vi "detect modules.vi"() -> (0 "error out":errorcluster, 1 "device models":string[](array[string]), 2 "passed?":bool)   [LabVIEW 2014, in "tests.lvlib"]
uses:
  tests.lvlib
  classes/Device/FG action.ctl
  classes/SysCfg Device/SysCfg Device.lvclass
  classes/Controller/Controller.lvclass
  classes/Chassis/Chassis.lvclass
  classes/Device/Device.lvclass
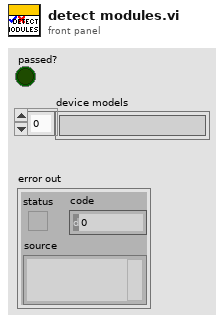
[diagram p1: front panel]
types:
  T1 = typedef "SMI.lvlib/Device.lvclass/FG action.ctl" = enum16{"get", "set"}
  T2 = typedef "SMI.lvlib/Device.lvclass/login credentials.ctl" = cluster{"device class":string, "hostname":string, "IP address":string, "username":string, "password":string}
  T3 = typedef "SMI.lvlib/Chassis.lvclass/chassis and module information.ctl" = cluster{"chassis":T4, "modules":T5[]}
  T4 = typedef "SMI.lvlib/Chassis.lvclass/chassis information.ctl" = cluster{"resource name":string, "vendor name":string, "product name":string, "product ID":u16, "serial number":string, "number of slots":i32, "device class":string}
  T5 = typedef "SMI.lvlib/Module.lvclass/module information.ctl" = cluster{"vendor name":string, "product name":string, "product ID":u16, "serial number":string}
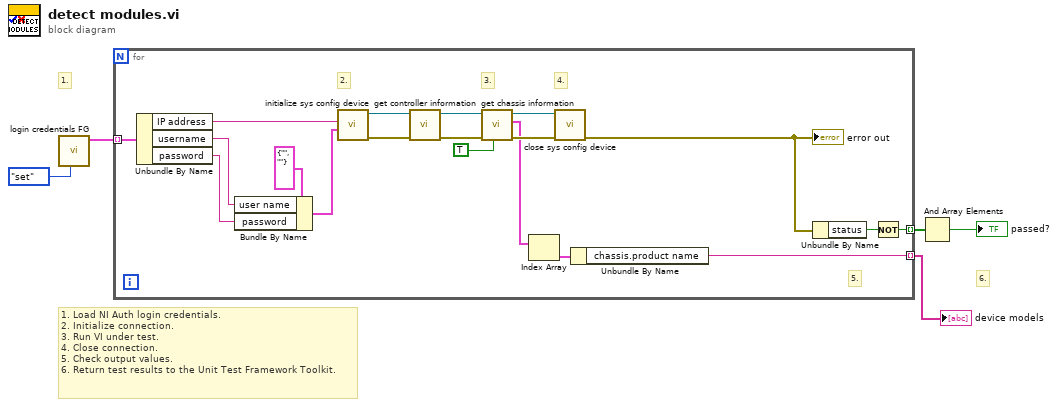
[diagram p0: block diagram]
diagram:
  # "1."
  # "6."
  # "1. Load NI Auth login credentials.\n2. Initialize connection.\n3. Run VI under test.\n4. Close connection.\n5. Check output values.\n6. Return test results to the Unit Test Framework Toolkit."
  n1 = call "login credentials FG.vi"("FG action"=FG_action."set") -> ("login credentials"=w3:T2[])  [unwired: 9 in, 1 out]
  n2 = for {
    tunnel: [w22] -> w4 mode=indexing
    tunnel: w3 -> [w13] mode=indexing
    tunnel: [w6] -> w2 mode=indexing
    # "4."
    # "2."
    # "3."
    # "5."
    n3 = Unbundle By Name(w13) -> ("IP address"=w12:string, "username"=w10:string, "password"=w11:string)
    n4 = Bundle By Name(cluster=cluster{"user name":string, "password":string} {"user name"="", "password"=""} ("login"), "user name"=w10, "password"=w11) -> (w14:cluster{"user name":string, "password":string})
    n5 = call "initialize sys config device.vi"("login"=w14, "IP address (localhost)"=w12) -> ("error out"=w24:errorcluster, "controller out"=w23:refnum<class "Controller.lvclass">)  [unwired: 8 in]
    n6 = call "get controller information.vi"("error in"=w24, "controller in"=w23) -> ("error out"=w21:errorcluster, "controller out"=w19:refnum<class "Controller.lvclass">)  [unwired: 7 in, 1 out]
    n7 = call "get chassis information.vi"("detect modules (T)"=TRUE, "error in"=w21, "controller in"=w19) -> ("error out"=w20:errorcluster, "local chassis"=w8:T3[], "controller out"=w18:refnum<class "Controller.lvclass">)  [unwired: 5 in, 1 out]
    n8 = Index Array(array=w8) -> (element=w7:T3)  [unwired: 1 in]
    n9 = call "close sys config device.vi"("error in"=w20, "controller in"=w18) -> ("error out"=w9:errorcluster)  [unwired: 8 in, 1 out]
    "error out" <- w9
    n10 = Unbundle By Name(w7) -> ("chassis.product name"=w6:string)
    n11 = Unbundle By Name(w9) -> ("status"=w17:bool)
    n12 = Not(x=w17) -> (.not. x?=w22:bool)
  }
  "device models" <- w2
  n13 = And Array Elements(Boolean array=w4) -> (logical AND=→"passed?":bool)
